vi "Prepare Request Dispatch.vi"(0 "request":string, 1 "protocol version":string, 2 "Mcp-Method":string, 3 "Mcp-Name":string, 5 "accepted?":bool, 7 "status code":u16, 9 "Accept":string, 11 "error in":errorcluster) -> (4 "accepted out":bool, 6 "status code out":u16, 8 "stream?":bool, 15 "error out":errorcluster)   [LabVIEW 2020, in "MCP Server.lvlib"]
doc: "Decides, in Process HTTP Request.vi and before Handle MCP Request.vi, how an accepted HTTP POST is answered.\n\nLEGACY CANCELLATION: a single JSON-RPC notification {\"method\":\"notifications/cancelled\",\"params\":{\"requestId\":..}} (MCP 2025-06-18 and older) is recorded in Legacy Cancellations.vi and answered with 202 at once; Handle MCP Request.vi is not called. The running tools/call sees it through Report Progress.vi and Cancel Requested.vi. While a STREAMED tools/call runs this works at once, because Process HTTP Request.vi returns as soon as the stream is set up. While a non-streamed tools/call runs, the notification waits behind it (Process HTTP Request.vi handles one request at a time) and has no effect. Every dispatched request first clears its own id from Legacy Cancellations.vi, so a notification that arrived too late never cancels a later request that reuses the id.\n\nSTREAMING: stream? is TRUE for a tools/call with an id whose params._meta.progressToken is a string or a number, when the Accept header contains text/event-stream and Check Modern MCP Request.vi would not refuse it. Both eras. Then accepted out is FALSE so that the request is not handled synchronously; Start Streamed Request.vi handles it instead.\n\nEverything else passes through unchanged."
uses:
  MCP Server.lvlib
  c4749c5b-ef16-49b2-98b6-755d3eefe205.vi
  <vilib>/JDP Science/JSONtext/Next JSON Value.vi
  <vilib>/JDP Science/JSONtext/String Subset.vi
  <vilib>/JDP Science/JSONtext/Parsing/Advance past next JSON Value (inlined COPY).vi
  <vilib>/JDP Science/JSONtext/Parsing/Advance past whitespace.vi
  <vilib>/JDP Science/JSONtext/Parsing/Advance past String.vi
  <vilib>/JDP Science/JSONtext/Parsing/Advance past Number.vi
  <vilib>/JDP Science/JSONtext/Parsing/Advance past Line Ending.vi
  <vilib>/JDP Science/JSONtext/Parsing/Parse Full Path or Item Name.vi
  <vilib>/JDP Science/JSONtext/Parsing/Advance past Array.vi
  <vilib>/JDP Science/JSONtext/Parsing/Advance past Object.vi
  <vilib>/JDP Science/JSONtext/support/Error Cluster From Code.vi
  <vilib>/JDP Science/JSONtext/Offset/Find Item Locations by Path.vi
  <vilib>/JDP Science/JSONtext/JSON text to Variant.vi
  <vilib>/JDP Science/JSONtext/LVClass Serializer/JSONtext LVClass Serializer.lvclass
  <vilib>/JDP Science/JSONtext/JSONtext.lvlib
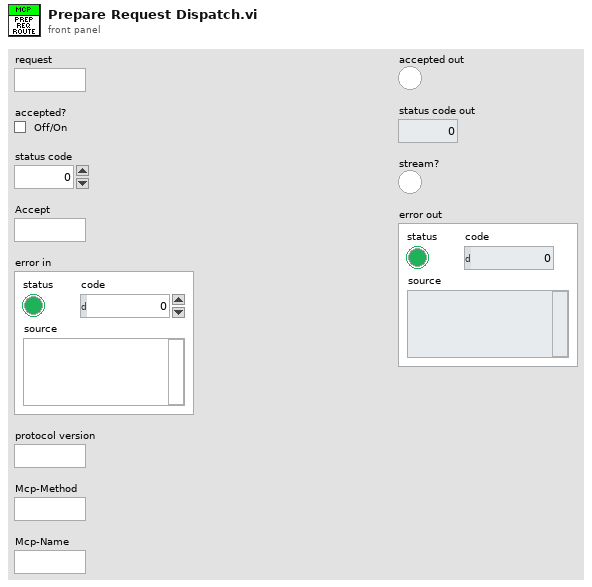
[diagram p1: front panel]
types:
  T1 = typedef "JSONtext.lvlib/JSON Value Type.ctl" = enum16{"Not a JSON Value", "JSON Object", "JSON Array", "String", "Number", "true", "false", "null"}
  T2 = typedef "MCP Server.lvlib/MCP Request Metadata.ctl" = cluster{"method":string, "id":string, "has id":bool, "modern":bool, "discover":bool, "batch":bool, "protocol version":string, "client capabilities":bool, "name or uri":string, "elicitation":bool, "input responses":string}
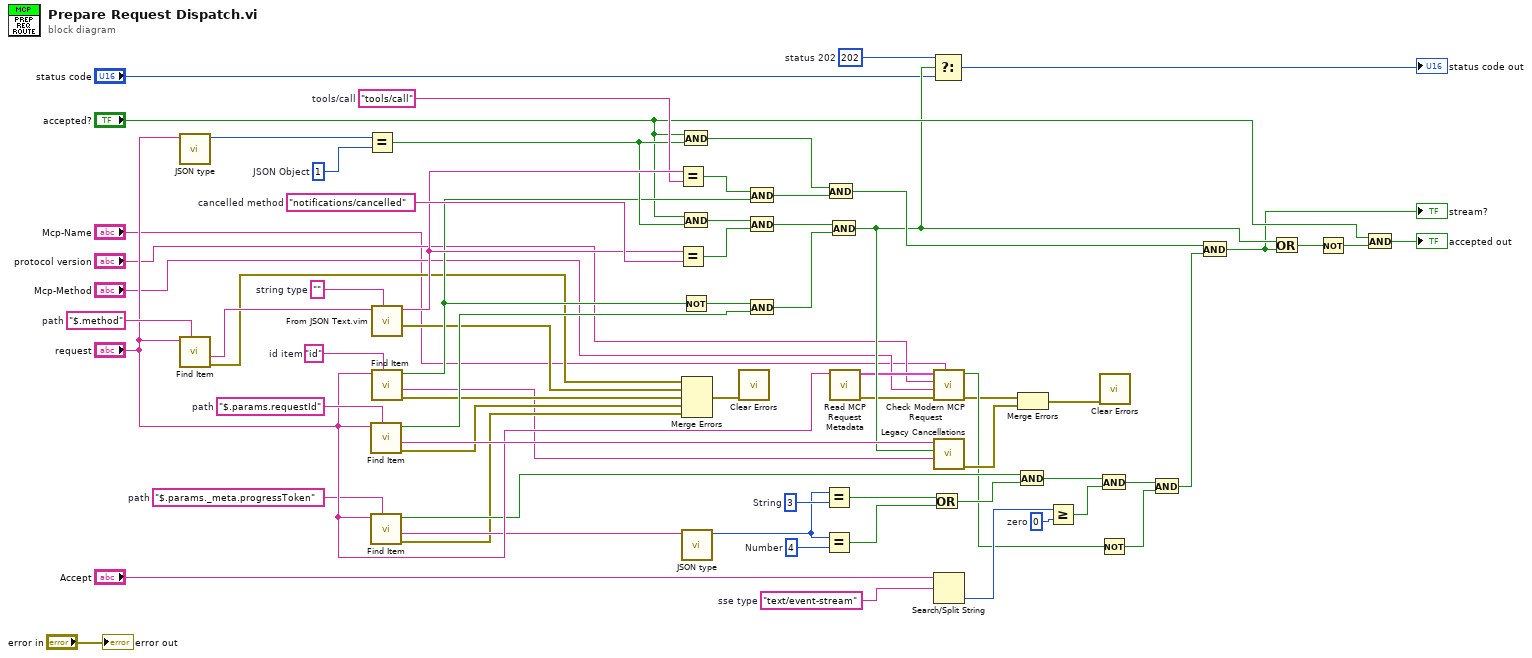
[diagram p0: block diagram]
diagram:
  w23 = u16 202  # status 202
  w38 = "tools/call"  # tools/call
  w40 = 0  # zero
  w42 = "text/event-stream"  # sse type
  w48 = u16 4  # Number
  w50 = u16 3  # String
  w52 = "$.params._meta.progressToken"  # path
  w61 = "notifications/cancelled"  # cancelled method
  w62 = "$.params.requestId"  # path
  w63 = "id"  # id item
  w64 = ""  # string type
  w66 = "$.method"  # path
  w67 = u16 1  # JSON Object
  n1 = call <vilib>:"JSON type.vi"("JSON"="request") -> ("JSON Value Type"=w68:T1)  [unwired: 9 in, 1 out]
  n2 = call <vilib>:"Find Item.vi"("$Path or Item Name"=w66, "JSON"="request") -> ("error out"=w20:errorcluster, "<JSON>"=w65:string)  [unwired: 6 in, 2 out]
  n3 = Equal?(x=w68, y=w67) -> (x = y?=w37:bool)
  n4 = call <vilib>:"Find Item.vi"("$Path or Item Name"=w62, "JSON"="request") -> ("error out"=w17:errorcluster, "<JSON>"=w54:string, "Found"=w57:bool)  [unwired: 6 in, 1 out]
  n5 = call <vilib>:"Find Item.vi"("$Path or Item Name"=w52, "JSON"="request") -> ("error out"=w16:errorcluster, "<JSON>"=w51:string, "Found"=w45:bool)  [unwired: 6 in, 1 out]
  n6 = call "From JSON Text.vim"("Data Type and Default Value"=w64, "JSON"=w65) -> ("error out"=w19:errorcluster, "Data out"=w39:string)  [unwired: 8 in]
  n7 = call <vilib>:"Find Item.vi"("$Path or Item Name"=w63, "JSON"="request") -> ("error out"=w18:errorcluster, "<JSON>"=w8:string, "Found"=w35:bool)  [unwired: 6 in, 1 out]
  n8 = Equal?(x=w39, y=w38) -> (x = y?=w36:bool)
  n9 = Equal?(x=w39, y=w61) -> (x = y?=w59:bool)
  n10 = And(x="accepted?", y=w37) -> (x .and. y?=w34:bool)
  n11 = And(x="accepted?", y=w37) -> (x .and. y?=w60:bool)
  n12 = Not(x=w35) -> (.not. x?=w58:bool)
  n13 = Merge Errors(w20, w19, w18, w17, w16) -> (w15:errorcluster)
  n14 = call <vilib>:"JSON type.vi"("JSON"=w51) -> ("JSON Value Type"=w49:T1)  [unwired: 9 in, 1 out]
  n15 = call <vilib>:"Clear Errors.vi"("error in (no error)"=w15) -> ()  [unwired: 5 in, 2 out]
  n16 = And(x=w36, y=w35) -> (x .and. y?=w33:bool)
  n17 = And(x=w60, y=w59) -> (x .and. y?=w56:bool)
  n18 = And(x=w58, y=w57) -> (x .and. y?=w55:bool)
  n19 = Equal?(x=w49, y=w50) -> (x = y?=w47:bool)
  n20 = Equal?(x=w49, y=w48) -> (x = y?=w46:bool)
  n21 = And(x=w34, y=w33) -> (x .and. y?=w28:bool)
  n22 = And(x=w56, y=w55) -> (x .and. y?=w22:bool)
  n23 = call "Read MCP Request Metadata.vi"("request"="request") -> ("error out"=w6:errorcluster, "MCP Request Metadata"=w7:T2)  [unwired: 9 in]
  n24 = Or(x=w47, y=w46) -> (x .or. y?=w44:bool)
  n25 = Select(t=w23, s=w22, f="status code") -> (s? t:f=→"status code out":u16)
  n26 = call "Check Modern MCP Request.vi"("Mcp-Name"="Mcp-Name", "error in"=w6, "Mcp-Method"="Mcp-Method", "protocol version"="protocol version", "MCP Request Metadata"=w7) -> ("error out"=w1:errorcluster, "refused"=w2:bool)  [unwired: 3 in, 2 out]
  n27 = call "Legacy Cancellations.vi"("started id"=w8, "add?"=w22, "request id"=w54) -> ("error out"=w14:errorcluster)  [unwired: 7 in, 1 out]
  n28 = Search/Split String(string="Accept", search string/char (-)=w42) -> (offset of match=w41:i32)  [unwired: 1 in, 2 out]
  n29 = And(x=w45, y=w44) -> (x .and. y?=w32:bool)
  n30 = Merge Errors(w1, w14) -> (w13:errorcluster)
  n31 = Greater Or Equal?(x=w41, y=w40) -> (x >= y?=w31:bool)
  n32 = And(x=w32, y=w31) -> (x .and. y?=w30:bool)
  n33 = Not(x=w2) -> (.not. x?=w29:bool)
  n34 = call <vilib>:"Clear Errors.vi"("error in (no error)"=w13) -> ()  [unwired: 5 in, 2 out]
  n35 = And(x=w30, y=w29) -> (x .and. y?=w27:bool)
  n36 = And(x=w28, y=w27) -> (x .and. y?=w10:bool)
  "stream?" <- w10
  n37 = Or(x=w22, y=w10) -> (x .or. y?=w26:bool)
  n38 = Not(x=w26) -> (.not. x?=w24:bool)
  n39 = And(x="accepted?", y=w24) -> (x .and. y?=→"accepted out":bool)
  "error out" <- "error in"
